vi "ASD Signal BL estimation VI.vi"(8 "R Peak location":i32[](array[numeric]), 11 "Estimated BL":dbl[](array[numeric])) -> (3 "Signal location BL":dbl[](array[numeric]))   [LabVIEW 2018]
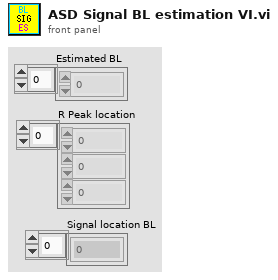
[diagram p1: front panel]
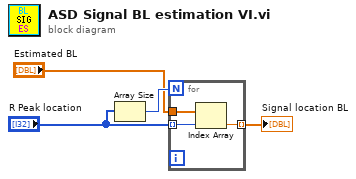
[diagram p0: block diagram]
diagram:
  n1 = Array Size(array="R Peak location") -> (size(s)=w4:i32)
  n2 = for {
    N: w4 -> [_]
    tunnel: "Estimated BL" -> [w7]
    tunnel: "R Peak location" -> [w6] mode=indexing
    tunnel: [w5] -> w1 mode=indexing
    n3 = Index Array(array=w7, index=w6) -> (element=w5:dbl)
  }
  "Signal location BL" <- w1
